vi "Test Serialize Clusters.vi"(8 "error in (no error)":errorcluster) -> (0 "error out":errorcluster)   [LabVIEW 2013]
uses:
  src/Serializer/JSON Serializer/JSON Serializer.lvclass
  <userlib>/_OpenG.lib/lvdata/lvdata.llb/Array of VData to VCluster__ogtk.vi
  <vilib>/addons/_JKI Toolkits/Caraya/classes/Test/Test.lvclass
  <vilib>/addons/_JKI Toolkits/Caraya/classes/Assert/Assert.lvclass
  src/JKI JSON Serialization.lvlib
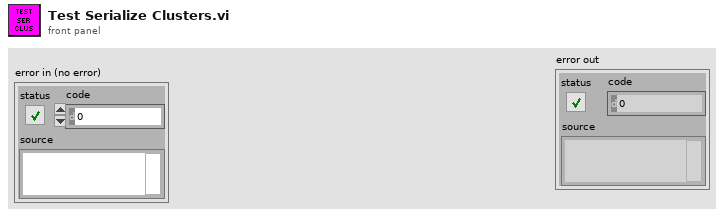
[diagram p1: front panel]
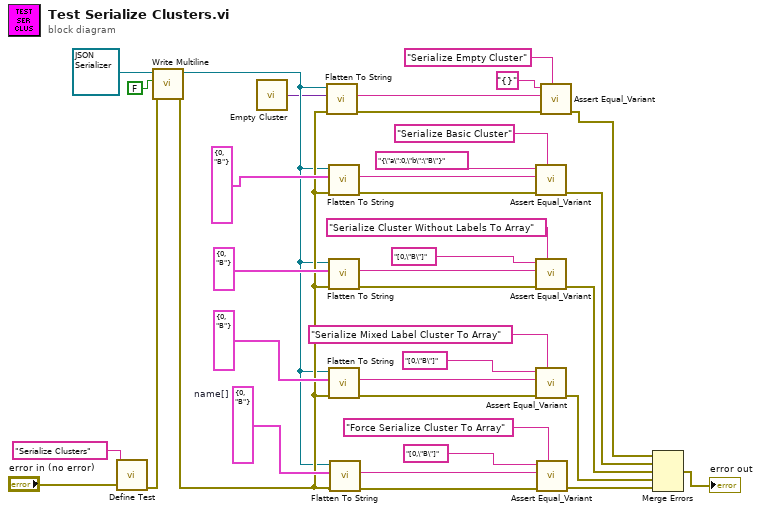
[diagram p0: block diagram]
diagram:
  w12 = cluster{"a":i32, "b":string} {"a"=0, "b"="B"}  # name[]
  n1 = call <vilib>:"Define Test.vi"("error in (no error)"="error in (no error)", "Label (VI Title)"="Serialize Clusters") -> ("error out"=w23:errorcluster)  [unwired: 9 in]
  n2 = call-dynamic "Write Multiline.vi"("error in (no error)"=w23, "Multiline"=FALSE, "JSON Serializer in"=refnum<class "JSON Serializer.lvclass"> refnum ("JKI JSON Serialization.lvlib:JSON Serializer.lvclass")) -> ("error out"=w8:errorcluster, "JSON Serializer out"=w7:refnum<class "JSON Serializer.lvclass">)  [unwired: 7 in]
  n3 = call "Empty Cluster.vi"() -> ("Empty Cluster"=w6:variant)
  n4 = call-dynamic "Flatten To String.vi"("error in (no error)"=w8, "Variant"=w6, "JSON Serializer in"=w7) -> ("error out"=w5:errorcluster, "String"=w3:string)  [unwired: 6 in, 1 out]
  n5 = call-dynamic "Flatten To String.vi"("error in (no error)"=w8, "Variant"=cluster{"a":i32, "b":string} {"a"=0, "b"="B"}, "JSON Serializer in"=w7) -> ("error out"=w33:errorcluster, "String"=w32:string)  [unwired: 6 in, 1 out]
  n6 = call-dynamic "Flatten To String.vi"("error in (no error)"=w8, "Variant"=cluster{i32, string} {0, "B"}, "JSON Serializer in"=w7) -> ("error out"=w36:errorcluster, "String"=w35:string)  [unwired: 6 in, 1 out]
  n7 = call-dynamic "Flatten To String.vi"("error in (no error)"=w8, "Variant"=cluster{"a":i32, string} {"a"=0, "B"}, "JSON Serializer in"=w7) -> ("error out"=w21:errorcluster, "String"=w16:string)  [unwired: 6 in, 1 out]
  n8 = call-dynamic "Flatten To String.vi"("error in (no error)"=w8, "Variant"=w12, "JSON Serializer in"=w7) -> ("error out"=w13:errorcluster, "String"=w11:string)  [unwired: 6 in, 1 out]
  n9 = call <vilib>:"Assert Equal_Variant.vi"("Label"="Serialize Basic Cluster", "error in (no error)"=w33, "Y"=w32, "X"="{\"a\":0,\"b\":\"B\"}") -> ("error out"=w26:errorcluster)  [unwired: 7 in]
  n10 = call <vilib>:"Assert Equal_Variant.vi"("Label"="Serialize Cluster Without Labels To Array", "error in (no error)"=w36, "Y"=w35, "X"="[0,\"B\"]") -> ("error out"=w27:errorcluster)  [unwired: 7 in]
  n11 = call <vilib>:"Assert Equal_Variant.vi"("Label"="Serialize Mixed Label Cluster To Array", "error in (no error)"=w21, "Y"=w16, "X"="[0,\"B\"]") -> ("error out"=w28:errorcluster)  [unwired: 7 in]
  n12 = call <vilib>:"Assert Equal_Variant.vi"("Label"="Force Serialize Cluster To Array", "error in (no error)"=w13, "Y"=w11, "X"="[0,\"B\"]") -> ("error out"=w9:errorcluster)  [unwired: 7 in]
  n13 = call <vilib>:"Assert Equal_Variant.vi"("Label"="Serialize Empty Cluster", "error in (no error)"=w5, "Y"=w3, "X"="{}") -> ("error out"=w4:errorcluster)  [unwired: 7 in]
  n14 = Merge Errors(w4, w26, w27, w28, w9) -> (→"error out":errorcluster)
